vi "test_input_required_result_request_state.vi"(8 "error in":errorcluster) -> (0 "error out":errorcluster, 3 "text":string)   [LabVIEW 2020, in "Conformance MCP Server.lvlib"]
doc: "Conformance fixture (scenario input-required-result-request-state). Takes no arguments and asks the user \"Please confirm\" with Ask User.vi (key confirm, a form with the boolean ok). The server answers the first call with input_required and a requestState and checks that requestState on the retry before this VI runs again; with the accepted answer text is \"state-ok: confirmed\". Without an accepted answer it returns at once and text is \"not confirmed\"."
uses:
  Conformance MCP Server.lvlib
  src/MCP Server/MCP Server.lvlib
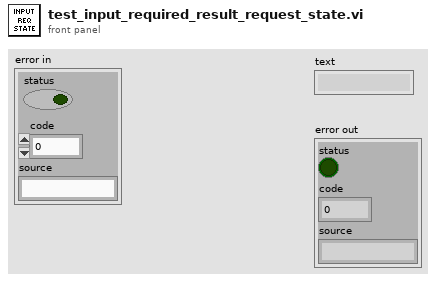
[diagram p1: front panel]
types:
  T1 = enum16{"accept", "decline", "cancel", "pending", "not supported"}
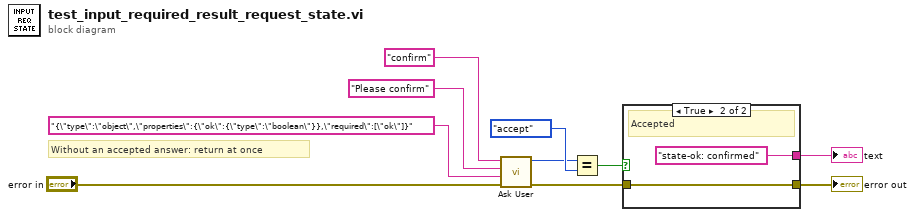
[diagram p0: block diagram]
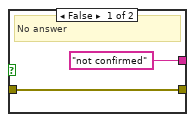
[diagram p2: hidden frame]
diagram:
  # "Without an accepted answer: return at once"
  n1 = call "Ask User.vi"("error in"="error in", "requestedSchema"="{\"type\":\"object\",\"properties\":{\"ok\":{\"type\":\"boolean\"}},\"required\":[\"ok\"]}", "message"="Please confirm", "key"="confirm") -> ("error out"=w6:errorcluster, "action"=w5:T1)  [unwired: 5 in, 1 out]
  n2 = Equal?(x=w5, y=T1."accept" ("accept")) -> (x = y?=w8:bool)
  n3 = case shown="True" w8 {
    tunnel: ["not confirmed" ("text") "state-ok: confirmed" ("text")] -> w9
    tunnel: w6 -> [w11 w13]
    tunnel: [w11 w13] -> w10
    frame False {
      # "No answer"
    }
    frame True {
      # "Accepted"
    }
  }
  "text" <- w9
  "error out" <- w10
